vi "pluto_bridge_test.vi"() -> ()   [LabVIEW 2026]
uses:
  <vilib>/Python/Open Venv Python Session.vi
panel:
  out "error out":errorcluster
  out "String":string
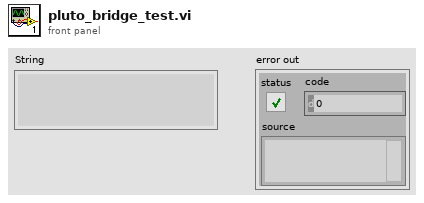
[diagram p1: front panel]
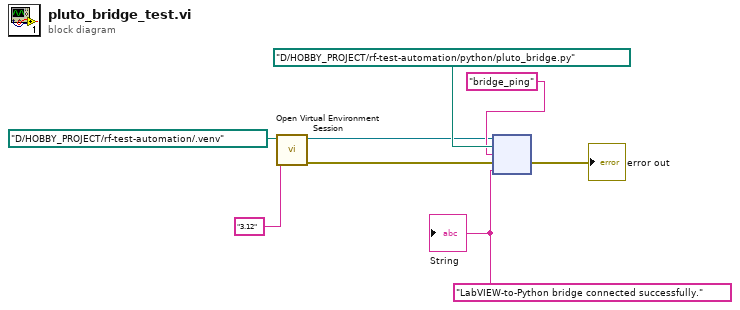
[diagram p0: block diagram]
diagram:
  w4 = "LabVIEW-to-Python bridge connected successfully."
  n1 = call-poly <vilib>:"Open Virtual Environment Session.vi"("Python version"="3.12", "Env path"=path "D:/HOBBY_PROJECT/rf-test-automation/.venv") -> ("error out"=w5:errorcluster, "session out"=w6:refnum<k35>)  [unwired: 8 in]
  n2 = node(w6, path "D:/HOBBY_PROJECT/rf-test-automation/python/pluto_bridge.py" ("module path"), "bridge_ping" ("function name"), w5, w4) -> (→"error out":errorcluster)  [unwired: 1 in, 3 out]
  "String" <- w4
